vi "Configure.vi"(8 "error in (no error)":errorcluster, 11 "ImageHandler:Varex-ImageHandler in":refnum<class "Varex-ImageHandler.lvclass">) -> (0 "error out":errorcluster, 3 "ImageHandler:Varex-ImageHandler out":refnum<class "Varex-ImageHandler.lvclass">)   [LabVIEW 2022 SP3, in "ImageHandler.lvlib" / "Varex-ImageHandler.lvclass"]
uses:
  Varex-ImageHandler.lvclass
  VarexWrapperLvLib/VarexWrapper.lvlib
panel:
  out "nHeight out":u16
  out "nWidth out":u16
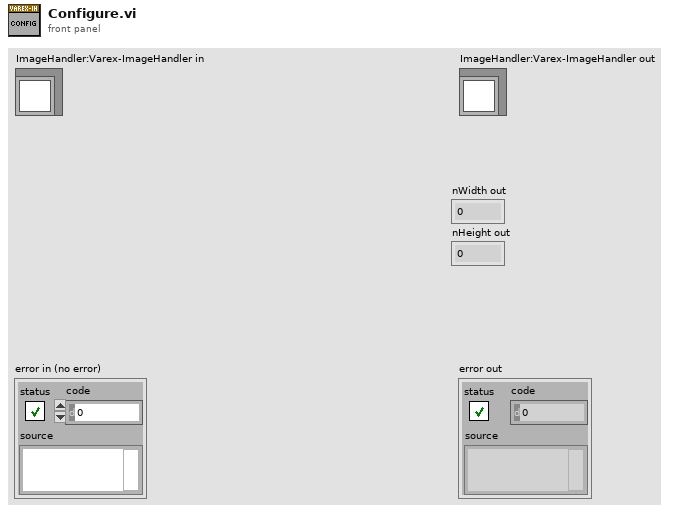
[diagram p1: front panel]
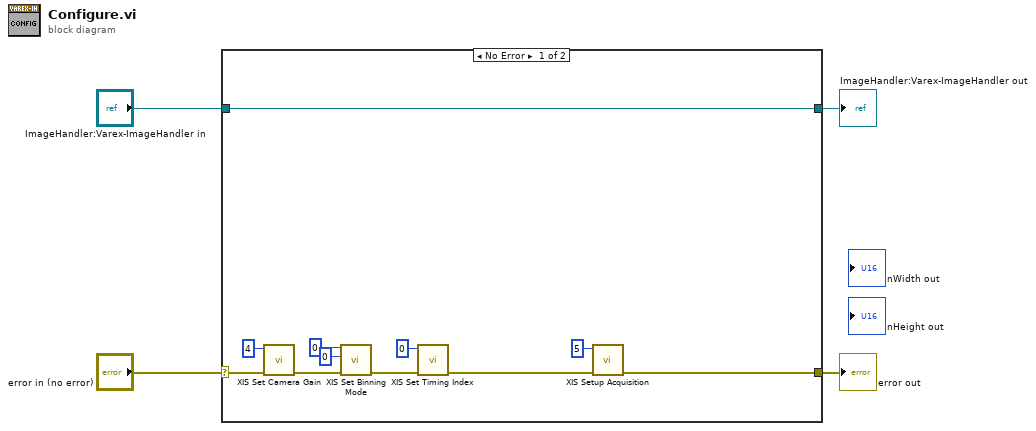
[diagram p0: block diagram]
diagram:
  n1 = case shown="No Error" "error in (no error)" {
    selector: "error in (no error)" -> [w14 w17]
    tunnel: [w10 w17] -> w3
    tunnel: [w15 w16] -> w1
    tunnel: "ImageHandler:Varex-ImageHandler in" -> [w15 w16]
    frame No Error {
      n2 = call "XIS Set Camera Gain.vi"("error in (no error)"=w14, "gainMode"=4) -> ("error out"=w12:errorcluster)  [unwired: 8 in, 1 out]
      n3 = call "XIS Set Binning Mode.vi"("error in (no error)"=w12, "accumulated"=0, "binningMode"=0) -> ("error out"=w11:errorcluster)  [unwired: 7 in, 1 out]
      n4 = call "XIS Set Timing Index.vi"("error in (no error)"=w11, "timingIndex"=0 ("timeMs")) -> ("error out"=w13:errorcluster)  [unwired: 8 in, 1 out]
      n5 = call "XIS Setup Acquisition.vi"("error in (no error)"=w13, "ringBuffCount"=5) -> ("error out"=w10:errorcluster)  [unwired: 8 in, 1 out]
    }
    frame Error {
    }
  }
  "error out" <- w3
  "ImageHandler:Varex-ImageHandler out" <- w1
